vi "WebDAV_DownloadAll.vi"(6 "IP myRIO":string="172.22.11.2", 9 "user":string, 10 "password":string, 11 "local file path":path) -> (0 "error out":errorcluster, 3 "dowloads":string[](array[string]))   [LabVIEW 2025]
uses:
  <vilib>/WebDAVClient/Advanced/Get File.vi
  <vilib>/WebDAVClient/NI_WebDAV.lvlib
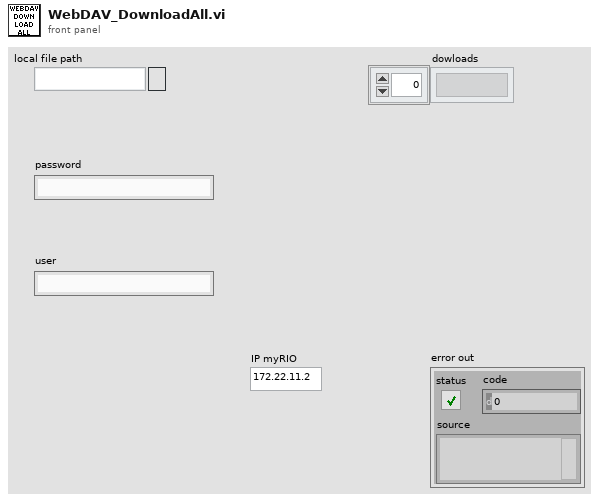
[diagram p1: front panel]
types:
  T1 = typedef "NI_WebDAV.lvlib/SessionHandle.ctl" = refnum<k1>
  T2 = typedef "NI_WebDAV.lvlib/FileInfo.ctl" = cluster{"type":string, "size":u64, "last modification":timestamp, "display name":string, "uri":string}
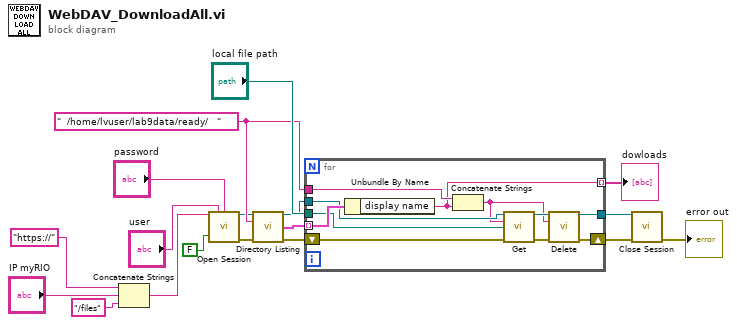
[diagram p0: block diagram]
diagram:
  w13 = "  /home/lvuser/lab9data/ready/   " ("relative uri")
  n1 = Concatenate Strings("https://" ("string"), "IP myRIO", "/files" ("string")) -> (w9:string)
  n2 = call <vilib>:"Open Session.vi"("host uri prefix"=w9, "username"="user", "password"="password", "verify server?"=FALSE) -> ("session handle out"=w8:T1, "error out"=w7:errorcluster)  [unwired: 10 in]
  n3 = call <vilib>:"Directory Listing.vi"("session handle"=w8, "relative uri"=w13, "error in (no error)"=w7) -> ("session handle out"=w12:T1, "file list"=w10:T2[], "error out"=w11:errorcluster)  [unwired: 9 in, 1 out]
  n4 = for {
    tunnel: w10 -> [w29] mode=indexing
    shift-right: [w21] -> w17
    shift-left: w11 -> [w26]
    tunnel: w12 -> [w28]
    tunnel: w13 -> [w20]
    tunnel: [w19] -> w14 mode=indexing
    tunnel: "local file path" -> [w27]
    tunnel: [w22] -> w16
    n5 = Unbundle By Name(w29) -> ("display name"=w19:string)
    n6 = Concatenate Strings(w20, w19) -> (w23:string)
    n7 = call-poly <vilib>:"Get.vi"("session handle"=w28, "relative uri"=w23, "local file path"=w27, "error in (no error)"=w26) -> ("session handle out"=w24:T1, "error out"=w25:errorcluster)  [unwired: 9 in, 1 out]
    n8 = call <vilib>:"Delete.vi"("session handle"=w24, "relative uri"=w23, "error in (no error)"=w25) -> ("session handle out"=w22:T1, "error out"=w21:errorcluster)  [unwired: 11 in]
  }
  "dowloads" <- w14
  n9 = call <vilib>:"Close Session.vi"("session handle"=w16, "error in (no error)"=w17) -> ("error out"=→"error out":errorcluster)  [unwired: 13 in]
